vi "RFH-save-common_format.vi"(5 "source":string, 7 "file path (use dialog)":path, 8 "error in (no error)":errorcluster, 10 "Common Format":T1) -> (0 "error out":errorcluster)   [LabVIEW 2020, in "RFH-Reflection_File_Handler.lvlib"]
doc: "Saves a Common Format cluster as a common-format file (dialog if no path) and writes the source text into the file."
uses:
  RFH-Reflection_File_Handler.lvlib
  RFH-common_data_format.ctl
  <vilib>/Utility/file.llb/Write Delimited Spreadsheet (DBL).vi
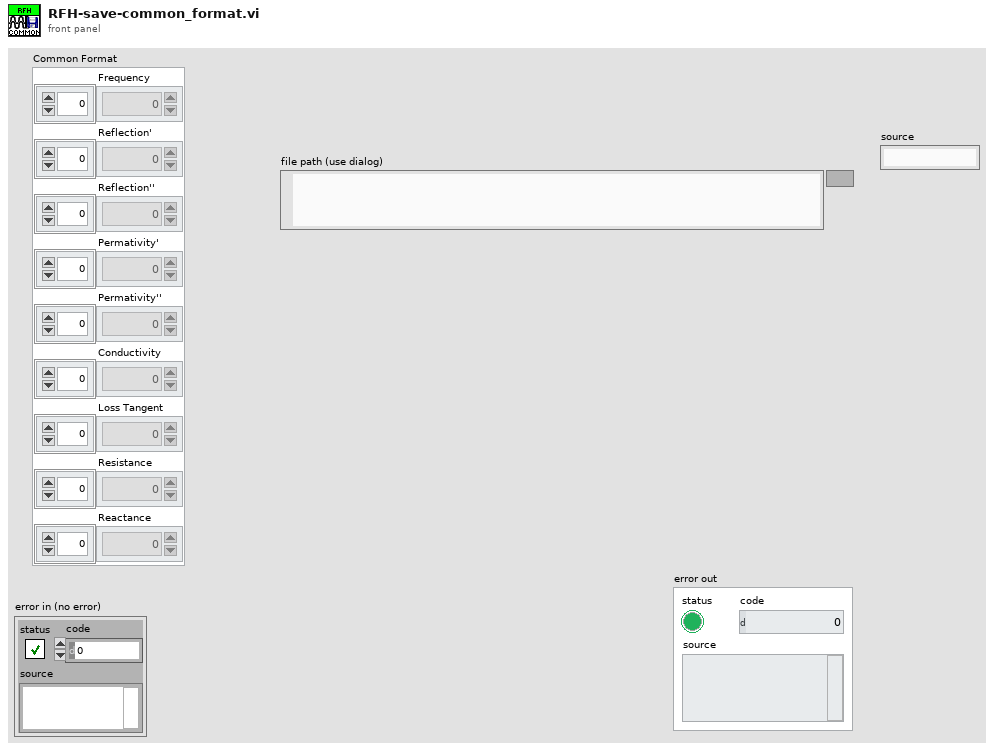
[diagram p1: front panel]
types:
  T1 = typedef "RFH-Reflection_File_Handler.lvlib/RFH-common_data_format.ctl" = cluster{"Frequency":dbl[], "Reflection'":dbl[], "Reflection''":dbl[], "Permativity'":dbl[], "Permativity''":dbl[], "Conductivity":dbl[], "Loss Tangent":dbl[], "Resistance":dbl[], "Reactance":dbl[]}
  T2 = enum16{"open", "replace", "create", "open or create", "replace or create", "replace or create with confirmation"}
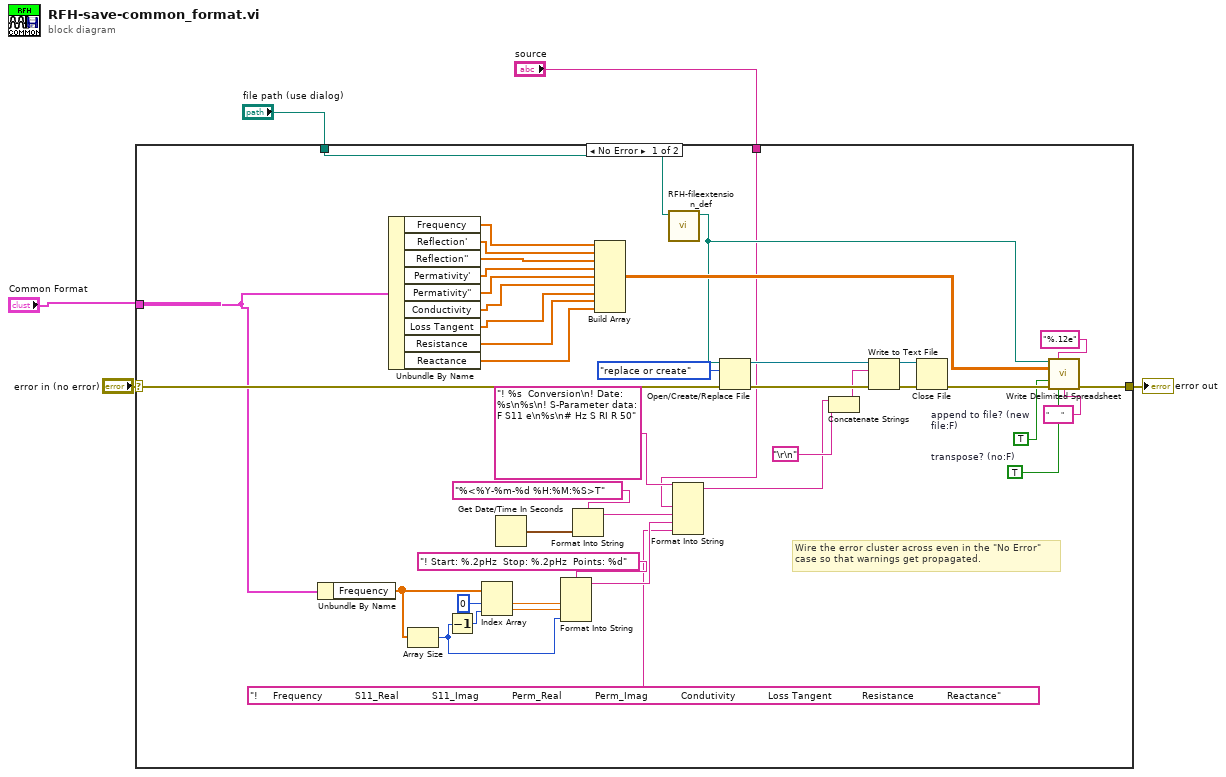
[diagram p0: block diagram]
diagram:
  n1 = case shown="No Error" "error in (no error)" {
    selector: "error in (no error)" -> [w22 w48]
    tunnel: [w14 w48] -> w3
    tunnel: "Common Format" -> [w15 _]
    tunnel: "file path (use dialog)" -> [w12 _]
    tunnel: "source" -> [w6 _]
    frame No Error {
      w29 = TRUE  # append to file? (new file:F)
      w31 = TRUE  # transpose? (no:F)
      # "Wire the error cluster across even in the \"No Error\"\ncase so that warnings get propagated."
      n2 = Unbundle By Name(w15) -> ("Frequency"=w21:dbl[])
      n3 = Unbundle By Name(w15) -> ("Frequency"=w25:dbl[], "Reflection'"=w27:dbl[], "Reflection''"=w26:dbl[], "Permativity'"=w24:dbl[], "Permativity''"=w13:dbl[], "Conductivity"=w10:dbl[], "Loss Tangent"=w9:dbl[], "Resistance"=w8:dbl[], "Reactance"=w7:dbl[])
      n4 = Array Size(array=w21) -> (size(s)=w16:i32)
      n5 = Decrement(x=w16) -> (x-1=w20:i32)
      n6 = Index Array(array=w21, index #1=0 ("index"), index #2=w20) -> (element #1=w18:dbl, element #2=w17:dbl)
      n7 = Get Date/Time In Seconds() -> (seconds since 1Jan1904=w38:timestamp)
      n8 = Format Into String(format string="! Start: %.2pHz  Stop: %.2pHz  Points: %d", w18, w17, w16) -> (resulting string=w34:string)  [unwired: 2 in, 1 out]
      n9 = Format Into String(format string="%<%Y-%m-%d %H:%M:%S>T", w38) -> (resulting string=w36:string)  [unwired: 2 in, 1 out]
      n10 = Build Array(w25, w27, w26, w24, w13, w10, w9, w8, w7) -> (w23:dbl[][])
      n11 = call "RFH-fileextension_def.vi"("Path in"=w12) -> ("Path with file extention"=w11:path)  [unwired: 9 in, 1 out]
      n12 = Format Into String(format string="! %s  Conversion\n! Date: %s\n%s\n! S-Parameter data: F S11 e\n%s\n# Hz S RI R 50" ("text"), w6, w36, w34, "!     Frequency           S11_Real           S11_Imag           Perm_Real           Perm_Imag           Condutivity           Loss Tangent          Resistance           Reactance" ("input 3")) -> (resulting string=w40:string)  [unwired: 2 in, 1 out]
      n13 = Open/Create/Replace File(file path (use dialog)=w11, error in=w22, operation (0:open)=T2."replace or create") -> (refnum out=w44:refnum<file>, error out=w45:errorcluster)  [unwired: 3 in, 1 out]
      n14 = Concatenate Strings(w40, "\r\n") -> (w41:string)
      n15 = Write to Text File(file (use dialog)=w44, text=w41, error in=w45) -> (refnum out=w46:refnum<file>, error out=w47:errorcluster)  [unwired: 1 in, 1 out]
      n16 = Close File(refnum=w46, error in=w47) -> (error out=w30:errorcluster)  [unwired: 1 out]
      n17 = call-poly <vilib>:"Write Delimited Spreadsheet.vi"("file path (dialog if empty)"=w11, "format (%.3f)"="%.12e", "2D data"=w23, "append to file? (new file:F)"=w29, "error in (no error)"=w30, "transpose? (no:F)"=w31, "delimiter (\\t)"="      " ("delimiter (\\t)")) -> ("error out"=w14:errorcluster)  [unwired: 7 in, 1 out]
    }
    frame Error {
    }
  }
  "error out" <- w3
